vi "Update Settings button colors.vi"(7 "Host in":T2, 8 "error in (no error)":errorcluster, 9 "Force Default Colors (F)":bool, 10 "Measurement UI Controls":T1, 11 "Settings in":T5) -> (0 "error out":errorcluster, 3 "Settings out":T5)   [LabVIEW 2021]
doc: "Change the colors of the boolean button according to 'Settings in' and 'Host in'. Consider whether the data log file will be overwritten: default colors when safe, red tint when overwriting. Otherwise, consider whether there are no IO resources: default colors when present, yellow tint when missing."
uses:
  Settings/Settings.ctl
  Acquisition/Hardware Configuration.ctl
  Acquisition/Channel Settings.ctl
  Acquisition/IO Device.ctl
  Acquisition/Sensor Type.ctl
  Interval Timer/Repeat Interval.ctl
  Interval Timer/Interval Length.ctl
  Interval Timer/Interval Token.ctl
  Acquisition/IO Context.ctl
  Acquisition/IO API.ctl
  Logging/Logging Configuration.ctl
  Logging/Logging Mode.ctl
  Diagnostics/Diagnostics Configuration.ctl
  controls/Graph Settings.ctl
  Acquisition/Host Resources.ctl
  Acquisition/Host Software Package.ctl
  Acquisition/Host IO Resource.ctl
  controls/UI Data.ctl
  Settings/Settings.lvlib
  Acquisition/Acquisition.lvlib
  Interval Timer/Interval Timer.lvlib
  Logging/Logging.lvlib
  Diagnostics/Diagnostics.lvlib
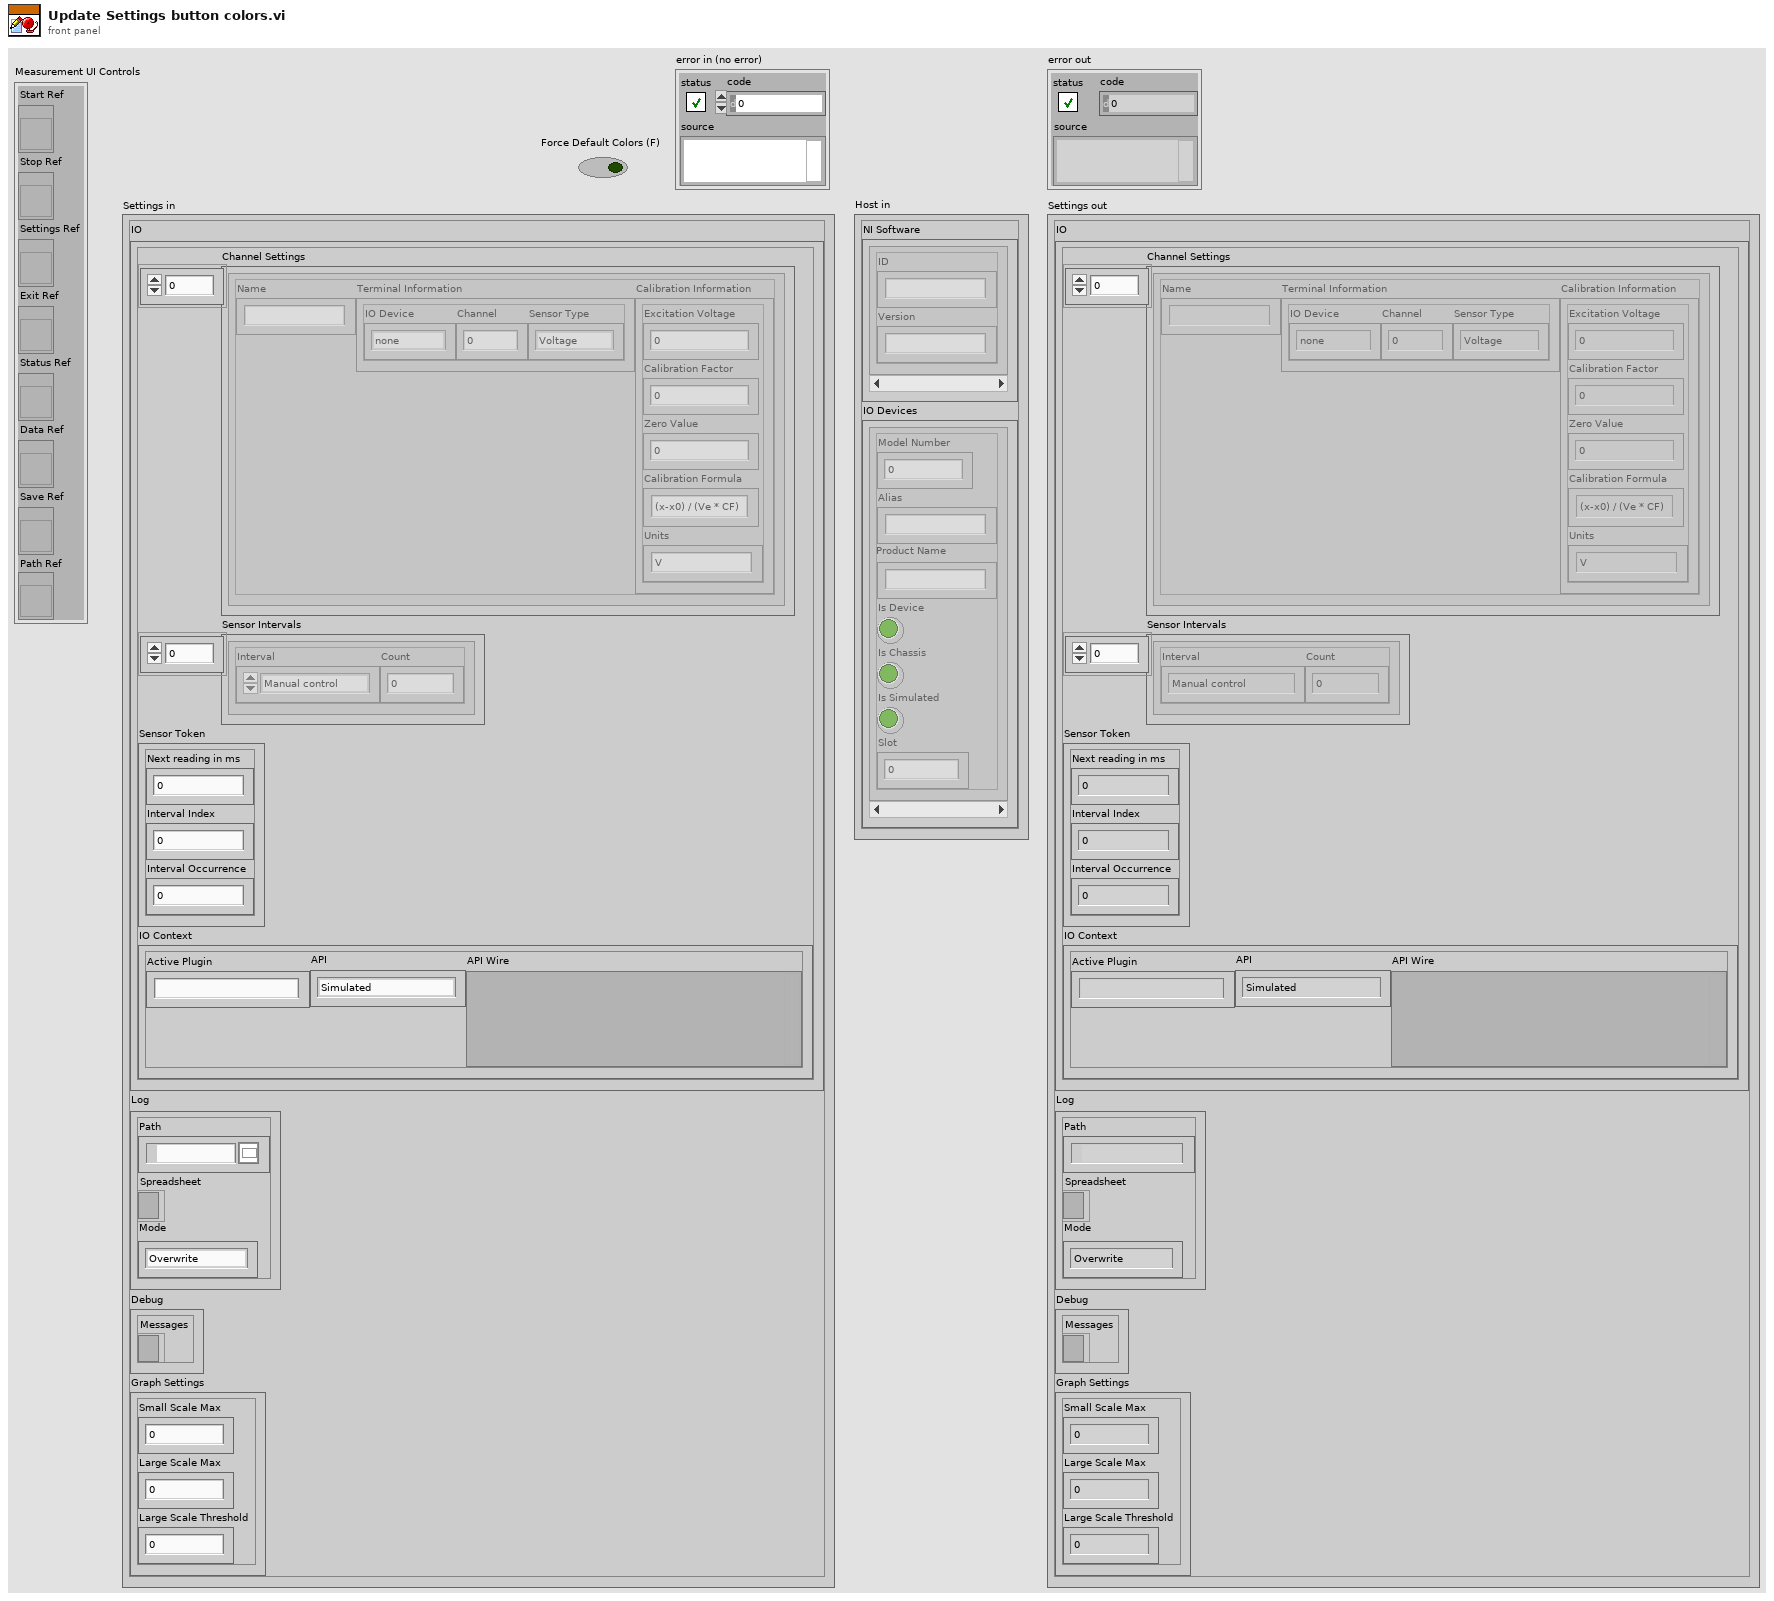
[diagram p1: front panel]
types:
  T1 = typedef "UI Data.ctl" = cluster{"Start Ref":refnum<vi>, "Stop Ref":refnum<vi>, "Settings Ref":refnum<vi>, "Exit Ref":refnum<vi>, "Status Ref":refnum<vi>, "Data Ref":refnum<vi>, "Save Ref":refnum<vi>, "Path Ref":refnum<vi>}
  T2 = typedef "Acquisition.lvlib/Host Resources.ctl" = cluster{"NI Software":T3[], "IO Devices":T4[]}
  T3 = typedef "Acquisition.lvlib/Host Software Package.ctl" = cluster{"ID":string, "Version":string}
  T4 = typedef "Acquisition.lvlib/Host IO Resource.ctl" = cluster{"Model Number":u32, "Alias":string, "Product Name":string, "Is Device":bool, "Is Chassis":bool, "Is Simulated":bool, "Slot":i32}
  T5 = typedef "Settings.lvlib/Settings.ctl" = cluster{"IO":T6, "Log":T15, "Debug":T17, "Graph Settings":T18}
  T6 = typedef "Acquisition.lvlib/Hardware Configuration.ctl" = cluster{"Channel Settings":T7[], "Sensor Intervals":T10[], "Sensor Token":T12, "IO Context":T13}
  T7 = typedef "Acquisition.lvlib/Channel Settings.ctl" = cluster{"Name":string, "Terminal Information":cluster{"IO Device":T8, "Channel":i32, "Sensor Type":T9}, "Calibration Information":cluster{"Excitation Voltage":dbl, "Calibration Factor":dbl, "Zero Value":dbl, "Calibration Formula":string, "Units":string}}
  T8 = typedef "Acquisition.lvlib/IO Device.ctl" = enum16{"none", "9219", "9401"}
  T9 = typedef "Acquisition.lvlib/Sensor Type.ctl" = enum16{"Voltage", "Load", "Pressure", "Encoder"}
  T10 = typedef "Interval Timer.lvlib/Repeat Interval.ctl" = cluster{"Interval":T11, "Count":i32}
  T11 = typedef "Interval Timer.lvlib/Interval Length.ctl" = enum16{"Manual control", "1 second", "10 seconds", "30 seconds", "60 seconds", "600 seconds", "1200 seconds", "3600 seconds"}
  T12 = typedef "Interval Timer.lvlib/Interval Token.ctl" = cluster{"Next reading in ms":u32, "Interval Index":i32, "Interval Occurrence":i32}
  T13 = typedef "Acquisition.lvlib/IO Context.ctl" = cluster{"Active Plugin":string, "API":T14, "API Wire":variant}
  T14 = typedef "Acquisition.lvlib/IO API.ctl" = enum16{"Simulated", "DAQmx"}
  T15 = typedef "Logging.lvlib/Logging Configuration.ctl" = cluster{"Path":path, "Spreadsheet":refnum<file>, "Mode":T16}
  T16 = typedef "Logging.lvlib/Logging Mode.ctl" = enum16{"Overwrite", "Append", "Create New"}
  T17 = typedef "Diagnostics.lvlib/Diagnostics Configuration.ctl" = cluster{"Messages":refnum<file>}
  T18 = typedef "Graph Settings.ctl" = cluster{"Small Scale Max":dbl, "Large Scale Max":dbl, "Large Scale Threshold":dbl}
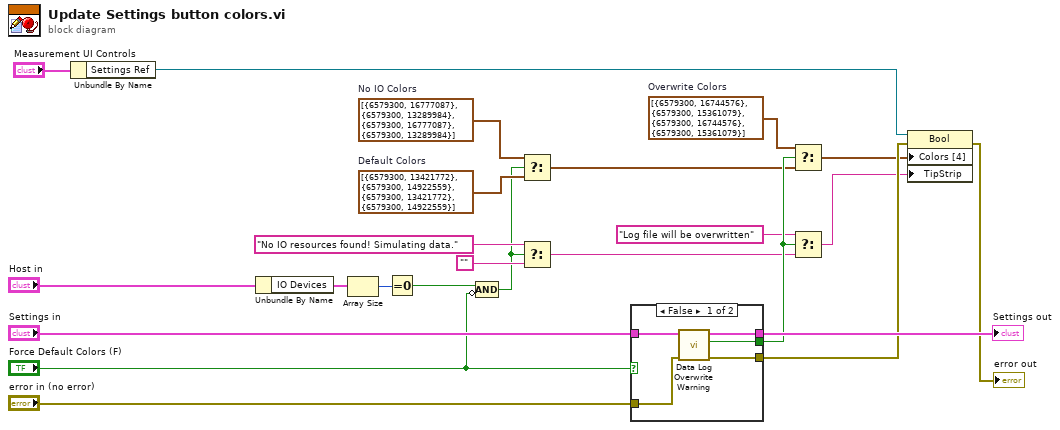
[diagram p0: block diagram]
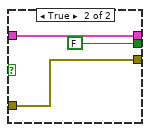
[diagram p2: hidden frame]
diagram:
  w9 = cluster{"Color Box":u32, "Color Box 2":u32}[] [{"Color Box"=6579300, "Color Box 2"=16777087}, {"Color Box"=6579300, "Color Box 2"=13289984}, {"Color Box"=6579300, "Color Box 2"=16777087}, {"Color Box"=6579300, "Color Box 2"=13289984}]  # No IO Colors
  w10 = cluster{"Color Box":u32, "Color Box 2":u32}[] [{"Color Box"=6579300, "Color Box 2"=13421772}, {"Color Box"=6579300, "Color Box 2"=14922559}, {"Color Box"=6579300, "Color Box 2"=13421772}, {"Color Box"=6579300, "Color Box 2"=14922559}]  # Default Colors
  w21 = cluster{"Color Box":u32, "Color Box 2":u32}[] [{"Color Box"=6579300, "Color Box 2"=16744576}, {"Color Box"=6579300, "Color Box 2"=15361079}, {"Color Box"=6579300, "Color Box 2"=16744576}, {"Color Box"=6579300, "Color Box 2"=15361079}]  # Overwrite Colors
  n1 = Unbundle By Name("Measurement UI Controls") -> ("Settings Ref"=w1:refnum<vi>)
  n2 = Unbundle By Name("Host in") -> ("IO Devices"=w13:T4[])
  n3 = Array Size(array=w13) -> (size(s)=w6:i32)
  n4 = Equal To 0?(x=w6) -> (x = 0?=w4:bool)
  n5 = Compound Arithmetic op=AND(w4, invert "Force Default Colors (F)") -> (w3:bool)
  n6 = Select(t=w9, s=w3, f=w10) -> (s? t:f=w8:cluster{"Color Box":u32, "Color Box 2":u32}[])
  n7 = Select(t="No IO resources found! Simulating data.", s=w3, f="") -> (s? t:f=w7:string)
  n8 = case shown="False" "Force Default Colors (F)" {
    tunnel: "Settings in" -> [w29 w30]
    tunnel: [w28 w30] -> w23
    tunnel: "error in (no error)" -> [w27 w31]
    tunnel: [w26 w31] -> w20
    tunnel: [w25 FALSE ("Overwrite Warning?")] -> w17
    frame False {
      n9 = call "Data Log Overwrite Warning.vi"("error in (no error)"=w27, "Settings in"=w29) -> ("error out"=w26:errorcluster, "Overwrite Warning?"=w25:bool, "Settings out"=w28:T5)  [unwired: 7 in]
    }
    frame True {
    }
  }
  "Settings out" <- w23
  n10 = Select(t=w21, s=w17, f=w8) -> (s? t:f=w18:cluster{"Color Box":u32, "Color Box 2":u32}[])
  n11 = Select(t="Log file will be overwritten", s=w17, f=w7) -> (s? t:f=w15:string)
  n12 = property class="Bool"(reference=w1, error in=w20, "Colors [4]"=w18, "TipStrip"=w15) -> (error out=→"error out":errorcluster)  [unwired: 1 out]
